vi "UDP Read.vi"(8 "错误输入（无错误）":errorcluster, 11 "连接ID":refnum<k16>) -> (0 "无错误":errorcluster, 2 "data out":string, 3 "连接ID输出":refnum<k16>)   [LabVIEW 2026, in "UI-距离测量.lvlib" / "UDP.lvlib"]
uses:
  UDP.lvlib
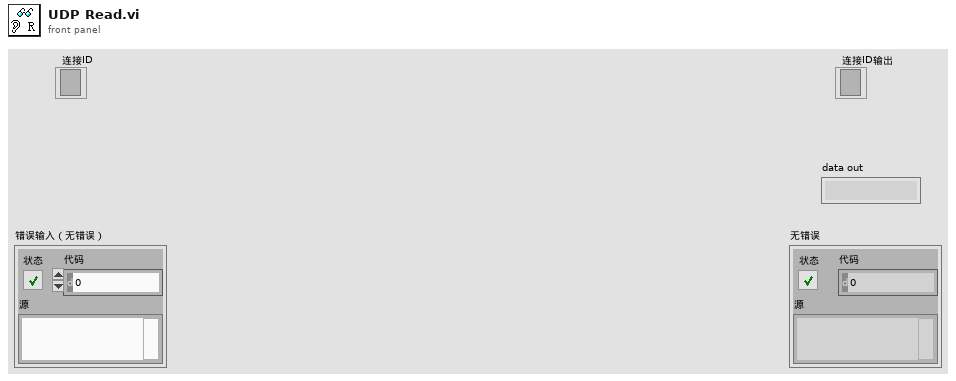
[diagram p1: front panel]
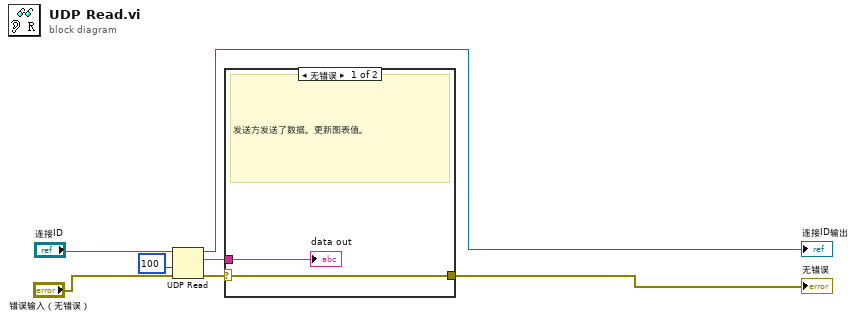
[diagram p0: block diagram]
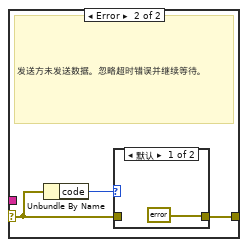
[diagram p2: hidden frame]
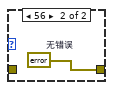
[diagram p3: hidden frame]
diagram:
  n1 = UDP Read(connection ID="连接ID", timeout ms (25000)=100, 8:"错误输入（无错误）") -> (data out=w6:string, error out=w5:errorcluster, 3:→"连接ID输出":refnum<k16>)  [unwired: 3 out]
  n2 = case shown="无错误" w5 {
    selector: w5 -> [w8 w11]
    tunnel: w6 -> [w9 _]
    tunnel: [w8 w10] -> w1
    frame No Error {
      # "发送方发送了数据。更新图表值。"
      "data out" <- w9
    }
    frame Error {
      # "发送方未发送数据。忽略超时错误并继续等待。"
      n3 = Unbundle By Name(w11) -> ("code"=w12:i32)
      n4 = case shown="默认" w12 {
        tunnel: w11 -> [_ _]
        tunnel: [errorcluster {"status"=FALSE, "code"=0, "source"=""} ("无错误") w14] -> w10
        frame Default {
        }
        frame 56 {
          w14 = errorcluster {"status"=FALSE, "code"=0, "source"=""}  # 无错误
        }
      }
    }
  }
  "无错误" <- w1
